vi "Get ILP2.vi"(7 "Color":T1, 8 "S (Distancia OLED-fotodiodo) cm":dbl, 11 "x (volts)":dbl) -> (2 "Luminancia (Cd/m2)":dbl, 3 "Iluminancia (lm/m2)":dbl)   [LabVIEW 2020]
uses:
  controls/Color --typedef.ctl
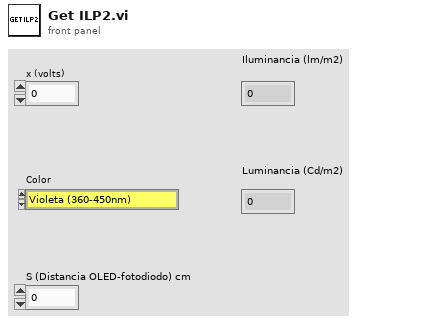
[diagram p1: front panel]
types:
  T1 = typedef "Color --typedef.ctl" = enum16{"Violeta (360-450nm)", "Azul (450-500nm)", "Verde(500-570nm)", "Amarillo (570-590nm)", "Naranja (600-610nm)", "Rojo (610-670nm)", "Blanco"}
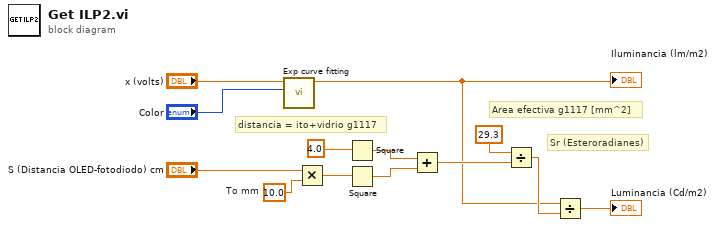
[diagram p0: block diagram]
diagram:
  w7 = 10.0  # To mm
  # "distancia = ito+vidrio g1117"
  # "Area efectiva g1117 [mm^2]"
  # "Sr (Esteroradianes)"
  n1 = call "Exp curve fitting.vi"("Color"="Color", "x (volts)"="x (volts)") -> ("y (Lux)"=w2:dbl)  [unwired: 9 in]
  "Iluminancia (lm/m2)" <- w2
  n2 = Multiply(x="S (Distancia OLED-fotodiodo) cm", y=w7) -> (x*y=w8:dbl)
  n3 = Square(x=4.0) -> (x^2=w13:dbl)
  n4 = Square(x=w8) -> (x^2=w12:dbl)
  n5 = Add(x=w13, y=w12) -> (x+y=w11:dbl)
  n6 = Divide(x=29.3 ("S"), y=w11) -> (x/y=w4:dbl)
  n7 = Divide(x=w2, y=w4) -> (x/y=→"Luminancia (Cd/m2)":dbl)
